vi "Write User Data.vi"(8 "error in (no error)":errorcluster, 10 "User Data":T2, 11 "Refnum in":T1) -> (0 "error out":errorcluster, 3 "Refnum out":T1)   [LabVIEW 2018]
uses:
  <vilib>/Utility/config.llb/Config Data RefNum.ctl
  <vilib>/TABOADA/Config Files Management/Config Files Management/config data--cluster.ctl
  <vilib>/TABOADA/Config Files Management/Config Files Management/Config Files Management.lvlib
  <vilib>/Utility/config.llb/NI_LVConfig.lvlib
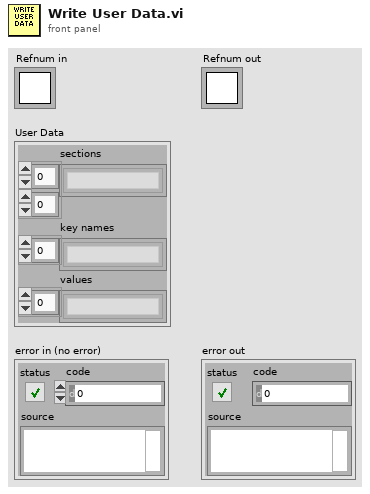
[diagram p1: front panel]
types:
  T1 = typedef "NI_LVConfig.lvlib/Config Data RefNum.ctl" = refnum<k1>
  T2 = typedef "Config Files Management.lvlib/config data--cluster.ctl" = cluster{"sections":string[][], "key names":string[], "values":string[]}
  T3 = enum16{"open", "replace", "create", "open or create", "replace or create", "replace or create with confirmation"}
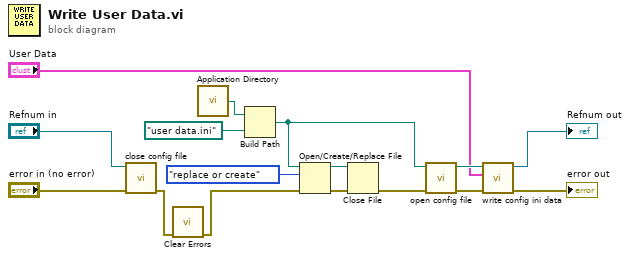
[diagram p0: block diagram]
diagram:
  n1 = call <vilib>:"close config file.vi"("error in (no error)"="error in (no error)", "Refnum in"="Refnum in") -> ("error out"=w2:errorcluster)  [unwired: 9 in]
  n2 = call <vilib>:"Clear Errors.vi"("error in (no error)"=w2) -> ("error out"=w1:errorcluster)  [unwired: 5 in, 1 out]
  n3 = call <vilib>:"Application Directory.vi"() -> ("Application Directory"=w6:path)
  n4 = Build Path(base path=w6, name or relative path=path "user data.ini") -> (appended path=w15:path)
  n5 = Open/Create/Replace File(file path (use dialog)=w15, error in=w1, operation (0:open)=T3."replace or create") -> (refnum out=w9:refnum<file>, error out=w10:errorcluster)  [unwired: 3 in, 1 out]
  n6 = Close File(refnum=w9, error in=w10) -> (error out=w14:errorcluster)  [unwired: 1 out]
  n7 = call <vilib>:"open config file.vi"("error in (no error)"=w14, "configuration file path"=w15) -> ("error out"=w12:errorcluster, "Refnum out"=w13:T1)  [unwired: 7 in, 1 out]
  n8 = call <vilib>:"write config ini data.vi"("error in (no error)"=w12, "data in"="User Data", "Refnum in"=w13) -> ("error out"=→"error out":errorcluster, "Refnum out"=→"Refnum out":T1)  [unwired: 7 in]
